vi "USBPT104Example.vi"() -> ()   [LabVIEW 2010]
panel:
  out "Ch4 Status":enum32{"Red", "Yellow", "Green"}(radio)
  out "Ch3 Status":enum32{"Red", "Yellow", "Green"}(radio)
  out "GetValue PICO_STATUS log":T1(array[cluster]) {"Hex Code" format="%x"}
  out "Ch2 Status":enum32{"Red", "Yellow", "Green"}(radio)
  out "Ch1 Status":enum32{"Red", "Yellow", "Green"}(radio)
  out "CH4 Value":dbl(slide)=nan min=-200.0 max=800.0 scale=0.0..115.0
  out "CH3 Value":dbl(slide)=nan min=-200.0 max=800.0 scale=0.0..10000.0
  out "CH2 Value":dbl(slide)=nan min=-200.0 max=800.0 scale=0.0..10000.0
  out "CH1 Value":dbl(slide)=nan min=-200.0 max=800.0 scale=-200.0..800.0
  in  "Channel Settings":T2={"CH1 # Wires"=4, "CH1 Measurement Type"=1, "CH2 # Wires"=2, "CH2 Measurement Type"=0, "CH3 # Wires"=2, "CH3 Measurement Type"=0, "CH4 # Wires"=2, "CH4 Measurement Type"=0} {"CH4 Measurement Type" items=["OFF", "PT100", "PT1000", "Resistance to 375 Ohms", "Resistance to 10 kOhms", "Differential to 115 mV", "Differential to 2500 mV", "Single-ended to 115 mV", "Single-ended to 2500 mV"]; "CH4 # Wires" items=["2"=2, "3"=3, "4"=4]; "CH3 Measurement Type" items=["OFF", "PT100", "PT1000", "Resistance to 375 Ohms", "Resistance to 10 kOhms", "Differential to 115 mV", "Differential to 2500 mV", "Single-ended to 115 mV", "Single-ended to 2500 mV"]; "CH3 # Wires" items=["2"=2, "3"=3, "4"=4]; "CH2 Measurement Type" items=["OFF", "PT100", "PT1000", "Resistance to 375 Ohms", "Resistance to 10 kOhms", "Differential to 115 mV", "Differential to 2500 mV", "Single-ended to 115 mV", "Single-ended to 2500 mV"]; "CH2 # Wires" items=["2"=2, "3"=3, "4"=4]; "CH1 Measurement Type" items=["OFF", "PT100", "PT1000", "Resistance to 375 Ohms", "Resistance to 10 kOhms", "Differential to 115 mV", "Differential to 2500 mV", "Single-ended to 115 mV", "Single-ended to 2500 mV"]; "CH1 # Wires" items=["2"=2, "3"=3, "4"=4]}
  out "Unit Info":T3
  in  "Connection":bool=TRUE
  in  "Use Serial Number":bool
  in  "Serial Number":string
  in  "IP Address:port number":string="192.168.1.30:6250"
  out "PT-104 Units":string
  in  "error in (no error)":errorcluster
  out "End time":timestamp=timestamp(-9593251199.456087 s since 1904-01-01)
  out "Start time":timestamp=timestamp(-9593251199.456087 s since 1904-01-01)
  out "error out":errorcluster
  in  "Update settings":bool
  in  "Stop":bool
  # "USB"
  # "Ethernet"
  # "Channel Status LED-\nYellow- Waiting/Off\nGreen- Read OK\nRed- Read Error"
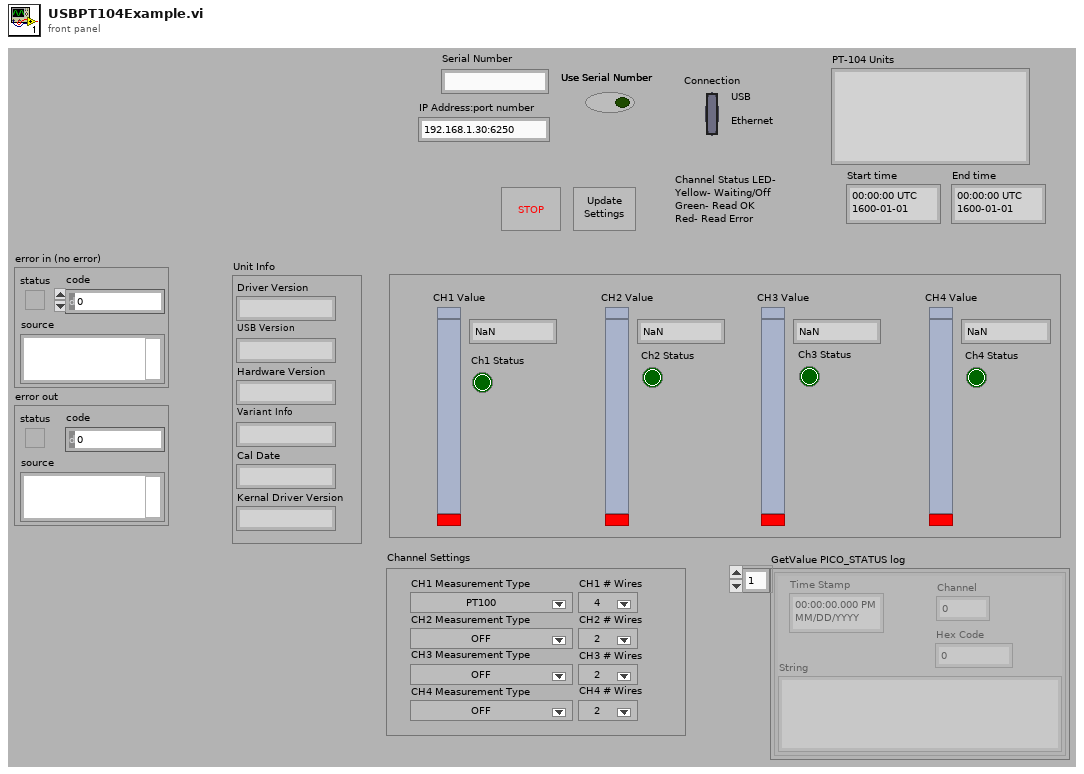
[diagram p1: front panel]
types:
  T1 = cluster{"Time Stamp":timestamp, "Hex Code":i32, "String":string, "Channel":i32}[]
  T2 = cluster{"CH1 # Wires":i16, "CH1 Measurement Type":i32, "CH2 # Wires":i16, "CH2 Measurement Type":i32, "CH3 # Wires":i16, "CH3 Measurement Type":i32, "CH4 # Wires":i16, "CH4 Measurement Type":i32}
  T3 = cluster{"Driver Version":string, "USB Version":string, "Hardware Version":string, "Variant Info":string, "Cal Date":string, "Kernal Driver Version":string, "NA":string, "NA 2":string, "NA":string, "NA 3":string, "NA 4":string, "NA 5":string, "NA 6":string, "NA 7":string, "NA 8":string}
  T4 = cluster{"seconds since 1Jan1904":timestamp, i32, "String":string, i32}[]
  T5 = cluster{"Channel Value":dbl, "Data Range:Maximum":dbl, "Scale.Range:Minimum":dbl}
  T6 = cluster{"seconds since 1Jan1904":timestamp, i32, "String":string, i32}
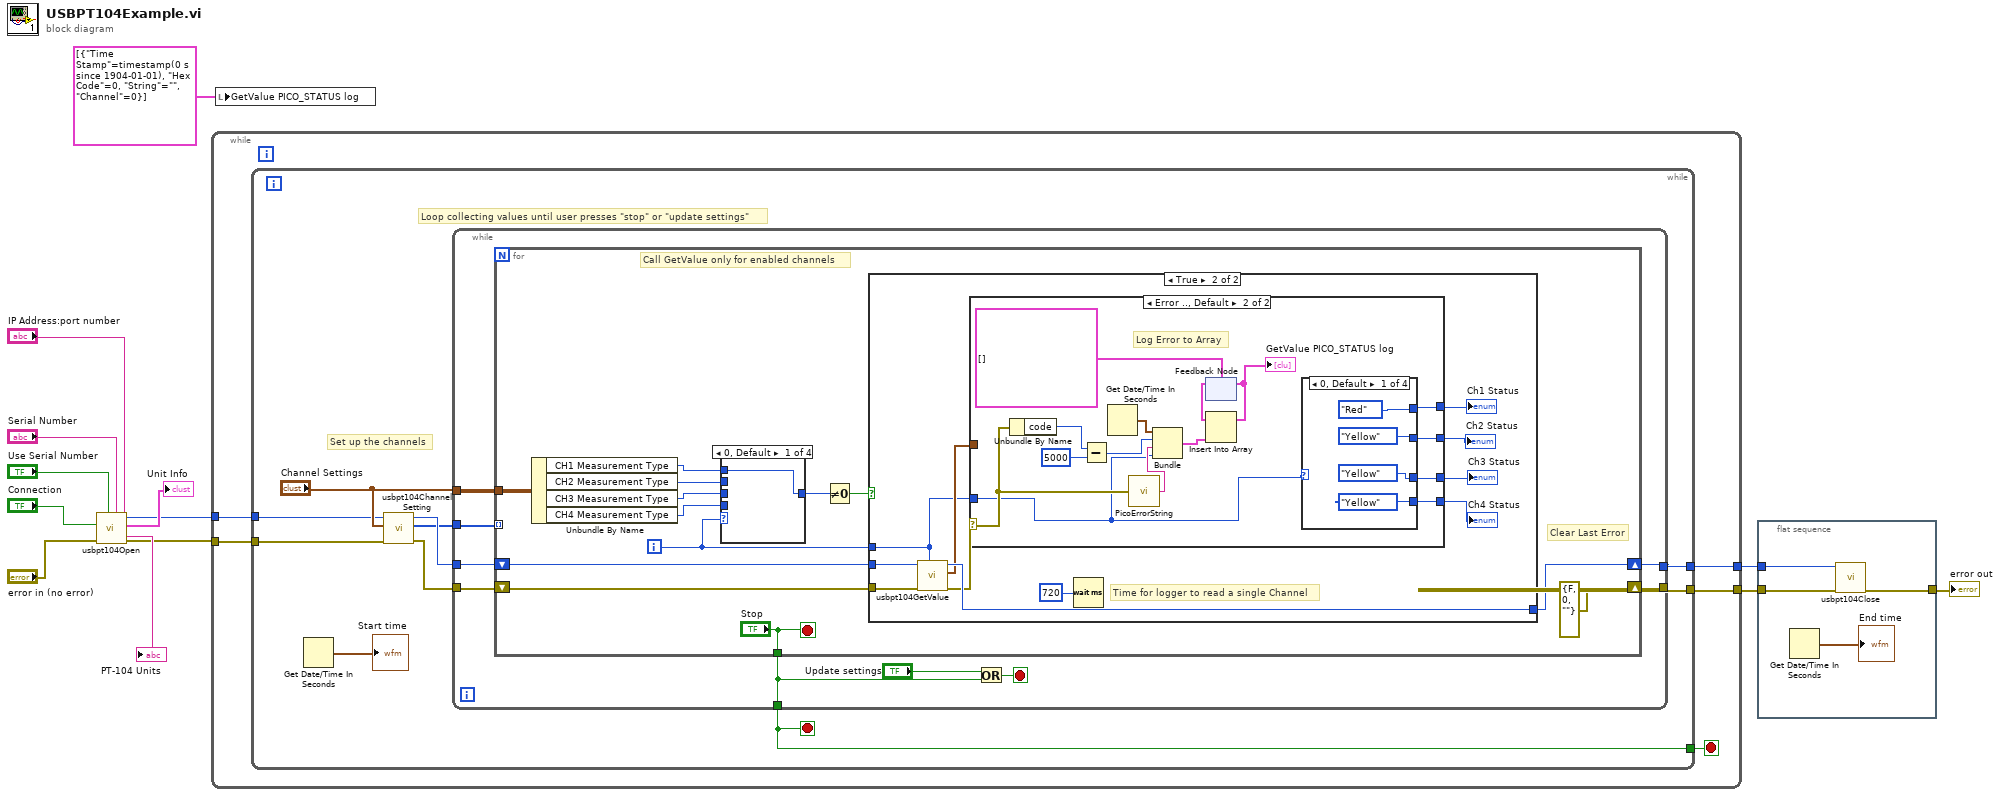
[diagram p0: block diagram]
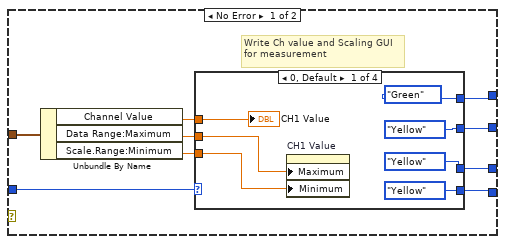
[diagram p6: hidden frame]
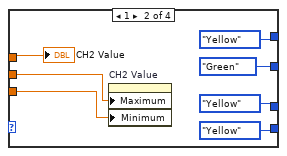
[diagram p7: hidden frame]
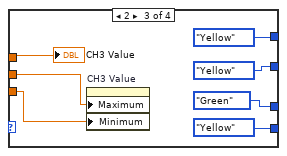
[diagram p8: hidden frame]
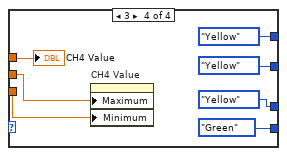
[diagram p9: hidden frame]
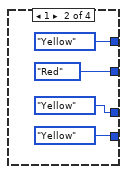
[diagram p10: hidden frame]
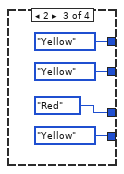
[diagram p11: hidden frame]
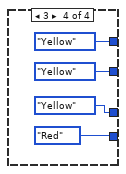
[diagram p12: hidden frame]
diagram:
  n1 = call "usbpt104Open.vi"("IP Address:port number"="IP Address:port number", "Serial Number"="Serial Number", "Use Serial Number"="Use Serial Number", "error in (no error)"="error in (no error)", "Connection"="Connection") -> ("error out"=w6:errorcluster, "Unit Info"=→"Unit Info":T3, "handle out"=w5:i16, "PT-104 Units"=→"PT-104 Units":string)  [unwired: 2 in, 1 out]
  n2 = while {
    tunnel: w6 -> [w18]
    tunnel: w5 -> [w17]
    tunnel: [w15] -> w4
    tunnel: [w14] -> w3
    stop <- w16 stop-if-true
    n3 = while {
      tunnel: [w28] -> w15
      tunnel: [w27] -> w14
      tunnel: [w23] -> w16
      tunnel: w18 -> [w22]
      tunnel: w17 -> [w21]
      stop <- w23 stop-if-true
      # "Loop collecting values until user presses \"stop\" or \"update settings\""
      # "Set up the channels"
      n4 = Get Date/Time In Seconds() -> (seconds since 1Jan1904=→"Start time":timestamp)
      n5 = call "usbpt104ChannelSetting.vi"("error in (no error)"=w22, "Channel Settings"="Channel Settings", "Handle In"=w21) -> ("error out"=w26:errorcluster, "Channel Enable Array"=w19:u8[], "Handle out"=w25:i16)  [unwired: 6 in]
      n6 = while {
        tunnel: w25 -> [w37]
        tunnel: w26 -> [w36]
        tunnel: [w33] -> w28
        tunnel: [w32] -> w27
        tunnel: [w30] -> w23
        tunnel: "Channel Settings" -> [w31]
        tunnel: w19 -> [w29]
        stop <- w35 stop-if-true
        n7 = for {
          shift-right: [errorcluster {"status"=FALSE, "code"=0, "source"=""} ("error out")] -> w33
          shift-left: w36 -> [w49]
          shift-right: [w46] -> w32
          shift-left: w37 -> [w50]
          tunnel: w31 -> [w44]
          tunnel: ["Stop"] -> w30
          tunnel: w29 -> [_] mode=indexing
          i -> [w45]
          stop <- "Stop" stop-if-true
          # "Clear Last Error"
          # "Call GetValue only for enabled channels"
          n8 = Unbundle By Name(w44) -> ("CH1 Measurement Type"=w43:i32, "CH2 Measurement Type"=w42:i32, "CH3 Measurement Type"=w41:i32, "CH4 Measurement Type"=w40:i32)
          n9 = case shown="0, Default" w45 {
            tunnel: [w51 w52 w53 w54] -> w47
            tunnel: w43 -> [w51 _ _ _]
            tunnel: w42 -> [_ w52 _ _]
            tunnel: w41 -> [_ _ w53 _]
            tunnel: w40 -> [_ _ _ w54]
            frame 0, Default {
            }
            frame 1 {
            }
            frame 2 {
            }
            frame 3 {
            }
          }
          n10 = Not Equal To 0?(x=w47) -> (x != 0?=w48:bool)
          n11 = case shown="True" w48 {
            tunnel: w50 -> [w55 w65]
            tunnel: w49 -> [_ w66]
            tunnel: [w55 w64] -> w46
            tunnel: w45 -> [_ w61]
            frame False {
            }
            frame True {
              # "Time for logger to read a single Channel"
              n12 = call "usbpt104GetValue.vi"("Channel"=w61, "error in (no error)"=w66, "handle in"=w65) -> ("error out"=w60:errorcluster, "Channel Data"=w62:T5, "handle out"=w64:i16)  [unwired: 6 in]
              n13 = case shown="Error .., Default" w60 {
                selector: w60 -> [_ w110]
                tunnel: w62 -> [w75 _]
                tunnel: w61 -> [w74 w107]
                tunnel: [w70 w109] -> w59
                tunnel: [w69 w108] -> w58
                tunnel: [w67 w106] -> w57
                tunnel: [w68 w105] -> w56
                frame No Error {
                  # "Write Ch value and Scaling GUI for measurement"
                  n14 = Unbundle By Name(w75) -> ("Channel Value"=w73:dbl, "Data Range:Maximum"=w72:dbl, "Scale.Range:Minimum"=w71:dbl)
                  n15 = case shown="0, Default" w74 {
                    tunnel: w73 -> [w82 w89 w96 w103]
                    tunnel: w72 -> [w81 w88 w95 w102]
                    tunnel: w71 -> [w80 w87 w94 w101]
                    tunnel: [enum32{"Red", "Yellow", "Green"}."Green" ("Select") enum32{"Red", "Yellow", "Green"}."Yellow" ("Select") enum32{"Red", "Yellow", "Green"}."Yellow" ("Select") enum32{"Red", "Yellow", "Green"}."Yellow" ("Select")] -> w70
                    tunnel: [enum32{"Red", "Yellow", "Green"}."Yellow" ("Select") enum32{"Red", "Yellow", "Green"}."Green" ("Select") enum32{"Red", "Yellow", "Green"}."Yellow" ("Select") enum32{"Red", "Yellow", "Green"}."Yellow" ("Select")] -> w69
                    tunnel: [enum32{"Red", "Yellow", "Green"}."Yellow" ("Select") enum32{"Red", "Yellow", "Green"}."Yellow" ("Select") enum32{"Red", "Yellow", "Green"}."Yellow" ("Select") enum32{"Red", "Yellow", "Green"}."Green" ("Select")] -> w68
                    tunnel: [enum32{"Red", "Yellow", "Green"}."Yellow" ("Select") enum32{"Red", "Yellow", "Green"}."Yellow" ("Select") enum32{"Red", "Yellow", "Green"}."Green" ("Select") enum32{"Red", "Yellow", "Green"}."Yellow" ("Select")] -> w67
                    frame 0, Default {
                      n16 = property on="CH1 Value" class="Slide (strict)"("Maximum"=w81, "Minimum"=w80) -> ()  [unwired: 2 in, 2 out]
                      "CH1 Value" <- w82
                    }
                    frame 1 {
                      n17 = property on="CH2 Value" class="Slide (strict)"("Maximum"=w88, "Minimum"=w87) -> ()  [unwired: 2 in, 2 out]
                      "CH2 Value" <- w89
                    }
                    frame 2 {
                      n18 = property on="CH3 Value" class="Slide (strict)"("Maximum"=w95, "Minimum"=w94) -> ()  [unwired: 2 in, 2 out]
                      "CH3 Value" <- w96
                    }
                    frame 3 {
                      n19 = property on="CH4 Value" class="Slide (strict)"("Maximum"=w102, "Minimum"=w101) -> ()  [unwired: 2 in, 2 out]
                      "CH4 Value" <- w103
                    }
                  }
                }
                frame Error, Default {
                  # "Log Error to Array"
                  n20 = Unbundle By Name(w110) -> ("code"=w111:i32)
                  n21 = Subtract(x=w111, y=5000) -> (x-y=w113:i32)
                  n22 = Get Date/Time In Seconds() -> (seconds since 1Jan1904=w115:timestamp)
                  n23 = call "PicoErrorString.vi"("error in"=w110) -> ("String"=w114:string)  [unwired: 2 in, 2 out]
                  n24 = Bundle("seconds since 1Jan1904"=w115, w113, "String"=w114, w107) -> (w118:T6)  [unwired: 1 in]
                  n25 = feedback #1(T4 []) -> (w116:T4)
                  n26 = Insert Into Array(array=w116, new element=w118) -> (w117:T4)  [unwired: 1 in]
                  "GetValue PICO_STATUS log" <- w117
                  n27 = feedback-in #1(w117) -> ()
                  n28 = case shown="0, Default" w107 {
                    tunnel: [enum32{"Red", "Yellow", "Green"}."Red" ("Select") enum32{"Red", "Yellow", "Green"}."Yellow" ("Select") enum32{"Red", "Yellow", "Green"}."Yellow" ("Select") enum32{"Red", "Yellow", "Green"}."Yellow" ("Select")] -> w109
                    tunnel: [enum32{"Red", "Yellow", "Green"}."Yellow" ("Select") enum32{"Red", "Yellow", "Green"}."Red" ("Select") enum32{"Red", "Yellow", "Green"}."Yellow" ("Select") enum32{"Red", "Yellow", "Green"}."Yellow" ("Select")] -> w108
                    tunnel: [enum32{"Red", "Yellow", "Green"}."Yellow" ("Select") enum32{"Red", "Yellow", "Green"}."Yellow" ("Select") enum32{"Red", "Yellow", "Green"}."Red" ("Select") enum32{"Red", "Yellow", "Green"}."Yellow" ("Select")] -> w106
                    tunnel: [enum32{"Red", "Yellow", "Green"}."Yellow" ("Select") enum32{"Red", "Yellow", "Green"}."Yellow" ("Select") enum32{"Red", "Yellow", "Green"}."Yellow" ("Select") enum32{"Red", "Yellow", "Green"}."Red" ("Select")] -> w105
                    frame 0, Default {
                    }
                    frame 1 {
                    }
                    frame 2 {
                    }
                    frame 3 {
                    }
                  }
                }
              }
              "Ch1 Status" <- w59
              "Ch2 Status" <- w58
              "Ch3 Status" <- w57
              "Ch4 Status" <- w56
              n29 = Wait (ms)(milliseconds to wait=u32 720) -> ()  [unwired: 1 out]
            }
          }
        }
        n30 = Or(x="Update settings", y=w30) -> (x .or. y?=w35:bool)
      }
    }
  }
  n31 = local write "GetValue PICO_STATUS log"(T1 [{"Time Stamp"=timestamp(0 s since 1904-01-01), "Hex Code"=0, "String"="", "Channel"=0}] ("GetValue PICO_STATUS log")) -> ()
  n32 = flat-sequence {
    tunnel: w4 -> [w138]
    tunnel: [w136] -> w2
    tunnel: w3 -> [w137]
    frame #0 {
      n33 = Get Date/Time In Seconds() -> (seconds since 1Jan1904=→"End time":timestamp)
      n34 = call "usbpt104Close.vi"("error in (no error)"=w138, "handle in"=w137) -> ("error out"=w136:errorcluster)  [unwired: 8 in, 1 out]
    }
  }
  "error out" <- w2
